vi "Read PJSA00339 File.vi"(11 "Path":path=path "D:/同步空间/曲线生成/原始曲线/2、帕捷--SA00339_2025041109.CSV") -> (3 "Data Series":T1[](array[typedef]))   [LabVIEW 2020, in "Data Viewer.lvlib"]
uses:
  Data Viewer.lvlib
  Data Serie--cluster.ctl
  File Type--enum.ctl
  <vilib>/Utility/file.llb/Read Delimited Spreadsheet (string).vi
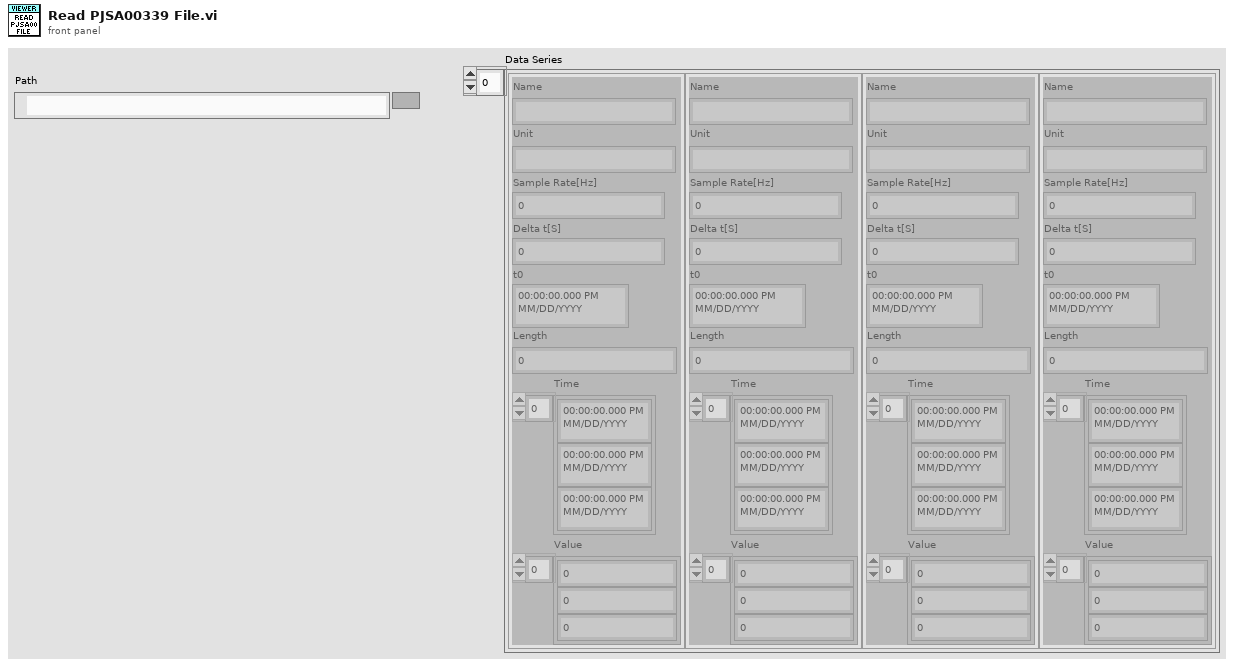
[diagram p1: front panel]
types:
  T1 = typedef "Data Viewer.lvlib/Data Serie--cluster.ctl" = cluster{"Name":string, "Unit":string, "Sample Rate[Hz]":dbl, "Delta t[S]":dbl, "t0":timestamp, "Length":i32, "Time":timestamp[], "Value":dbl[]}
  T2 = typedef "Data Viewer.lvlib/File Type--enum.ctl" = enum16{"伟思环境箱", "增达环境箱", "广五所环境箱", "无纸记录仪", "帕捷SA00339", "记录仪840", "记录仪8400", "记录仪MR888", "*.csv"}
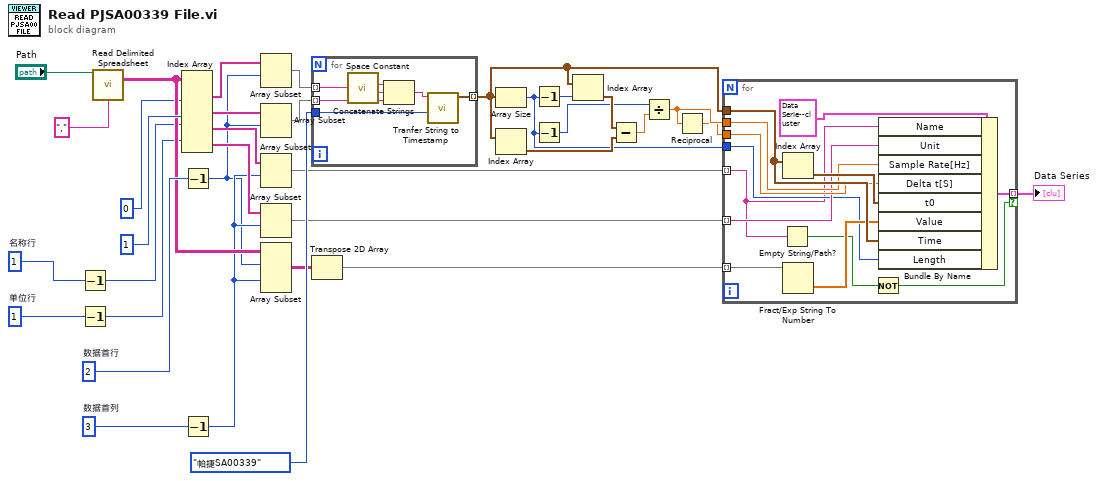
[diagram p0: block diagram]
diagram:
  w25 = 3  # 数据首列
  w26 = 2  # 数据首行
  w28 = 1  # 单位行
  w30 = 1  # 名称行
  n1 = Decrement(x=w30) -> (x-1=w10:i32)
  n2 = Decrement(x=w28) -> (x-1=w9:i32)
  n3 = call-poly <vilib>:"Read Delimited Spreadsheet.vi"("file path (dialog if empty)"="Path", "delimiter (\\t)"="," ("delimiter (\\t)")) -> ("all rows"=w11:string[][])  [unwired: 8 in, 5 out]
  n4 = Index Array(array=w11, index (col) #1=0 ("disabled index (col)"), index (col) #2=1 ("disabled index (col)"), index (row) #3=w10, index (row) #4=w9) -> (element #1=w4:string[], element #2=w33:string[], element #3=w29:string[], element #4=w27:string[])  [unwired: 4 in]
  n5 = Decrement(x=w26) -> (x-1=w5:i32)
  n6 = Decrement(x=w25) -> (x-1=w8:i32)
  n7 = Array Subset(array=w4, index=w5) -> (w3:string[])  [unwired: 1 in]
  n8 = Array Subset(array=w33, index=w5) -> (w32:string[])  [unwired: 1 in]
  n9 = Array Subset(array=w29, index=w8) -> (w23:string[])  [unwired: 1 in]
  n10 = Array Subset(array=w27, index=w8) -> (w22:string[])  [unwired: 1 in]
  n11 = Array Subset(array=w11, index (row)=w5, index (col)=w8) -> (w24:string[][])  [unwired: 2 in]
  n12 = for {
    tunnel: w32 -> [w37] mode=indexing
    tunnel: File_Type--enum."帕捷SA00339" ("File Type") -> [w40]
    tunnel: [w39] -> w20 mode=indexing
    tunnel: w3 -> [w38] mode=indexing
    n13 = call <vilib>:"Space Constant.vi"() -> ("String"=w36:string)
    n14 = Concatenate Strings(w38, w36, w37) -> (w35:string)
    n15 = call "Tranfer String to Timestamp.vi"("File Type"=w40, "String"=w35) -> ("time stamp"=w39:timestamp)  [unwired: 9 in]
  }
  n16 = Transpose 2D Array(2D array=w24) -> (transposed array=w21:string[][])
  n17 = Array Size(array=w20) -> (size(s)=w6:i32)
  n18 = Index Array(array=w20) -> (element=w17:timestamp)  [unwired: 1 in]
  n19 = Decrement(x=w6) -> (x-1=w19:i32)
  n20 = Decrement(x=w6) -> (x-1=w7:i32)
  n21 = Index Array(array=w20, index=w19) -> (element=w18:timestamp)
  n22 = Subtract(x=w18, y=w17) -> (x-y=w16:dbl)
  n23 = Divide(x=w7, y=w16) -> (x/y=w15:dbl)
  n24 = Reciprocal(x=w15) -> (1/x=w14:dbl)
  n25 = for {
    tunnel: w23 -> [w43] mode=indexing
    tunnel: w22 -> [w45] mode=indexing
    tunnel: w21 -> [w50] mode=indexing
    tunnel: w20 -> [w51]
    tunnel: w15 -> [w48]
    tunnel: w14 -> [w47]
    tunnel: [w46] -> w13 mode=indexing if=w41
    tunnel: w6 -> [w44]
    n26 = Empty String/Path?(string/path=w43) -> (empty?=w42:bool)
    n27 = Index Array(array=w51) -> (element=w52:timestamp)  [unwired: 1 in]
    n28 = Fract/Exp String To Number(string=w50) -> (number=w49:dbl[])  [unwired: 3 in, 1 out]
    n29 = Not(x=w42) -> (.not. x?=w41:bool)
    n30 = Bundle By Name(cluster=T1 {"Name"="", "Unit"="", "Sample Rate[Hz]"=0.0, "Delta t[S]"=0.0, "t0"=timestamp(0 s since 1904-01-01), "Length"=0, "Time"=[], "Value"=[]} ("Data Serie"), "Name"=w43, "Unit"=w45, "Sample Rate[Hz]"=w48, "Delta t[S]"=w47, "t0"=w52, "Value"=w49, "Time"=w51, "Length"=w44) -> (w46:T1)
  }
  "Data Series" <- w13
